vi "Test - Read Task Rows.vi"(8 "error in":errorcluster, 10 "Project ID":string, 11 "Data Folder":path) -> (0 "error out":errorcluster, 1 "Active":bool[](array[boolean]), 2 "Task Names":string[](array[string]), 3 "Project Store out":refnum<class "Project Store.lvclass">, 5 "Active Task IDs":string[](array[string]))   [LabVIEW 2026]
doc: "Test support for Test Task Rows.vi. Reads the data folder from disk with a fresh Initialize Stores.vi and returns one project's tasks as Project Task Rows.vi gives them (all tasks in Sort Order, split into Task Names and Active) plus the IDs of its active tasks from Task List.vi. Project Store out is the freshly read store, for a test that goes on to change it.\n\nInputs: Data Folder; Project ID; error in.\nOutputs: Project Store out; Task Names; Active; Active Task IDs; error out.\n\nGenerated by: Claude"
uses:
  Storage/Project Store/Project Store.lvclass
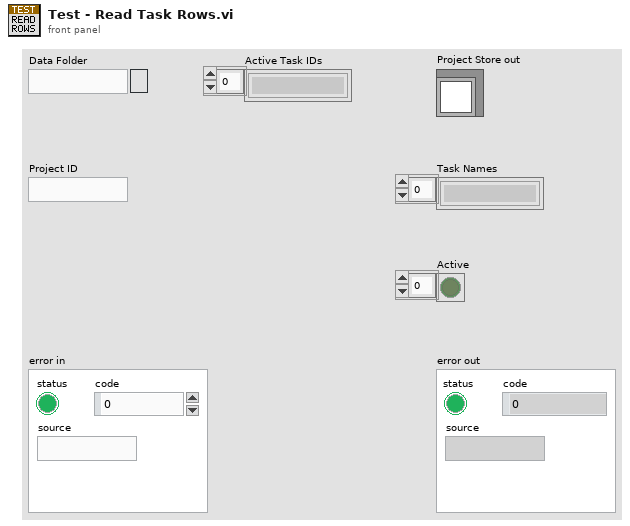
[diagram p1: front panel]
types:
  T1 = typedef "Task Edit Row.ctl" = cluster{"Task Name":string, "Active":bool}
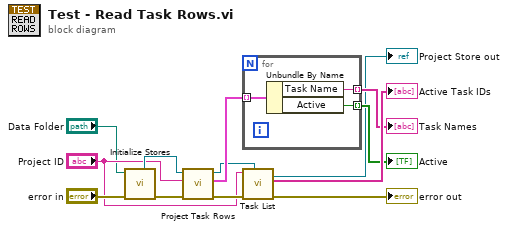
[diagram p0: block diagram]
diagram:
  n1 = call "Initialize Stores.vi"("error in"="error in", "Data Folder"="Data Folder") -> ("error out"=w9:errorcluster, "Project Store out"=w10:refnum<class "Project Store.lvclass">)  [unwired: 5 in, 3 out]
  n2 = call "Project Task Rows.vi"("error in"=w9, "Project ID"="Project ID", "Project Store in"=w10) -> ("error out"=w13:errorcluster, "Task Rows"=w12:T1[], "Project Store out"=w11:refnum<class "Project Store.lvclass">)  [unwired: 6 in]
  n3 = for {
    tunnel: w12 -> [w14] mode=indexing
    tunnel: [w15] -> w5 mode=indexing
    tunnel: [w16] -> w6 mode=indexing
    n4 = Unbundle By Name(w14) -> ("Task Name"=w15:string, "Active"=w16:bool)
  }
  "Task Names" <- w5
  "Active" <- w6
  n5 = call "Task List.vi"("Project Store in"=w11, "error in"=w13, "Project ID"="Project ID") -> ("error out"=→"error out":errorcluster, "Task IDs"=→"Active Task IDs":string[], "Project Store out"=→"Project Store out":refnum<class "Project Store.lvclass">)  [unwired: 5 in, 1 out]
